vi "Route MT8000A Command.vi"(8 "error in (no error)":errorcluster caption="에러 입력(에러 없음)", 10 "문자열":string, 11 "Instrument Manager 입력":refnum<class "Instrument Manager.lvclass">) -> (0 "error out":errorcluster caption="에러 출력", 3 "Instrument Manager 출력":refnum<class "Instrument Manager.lvclass">)   [LabVIEW 2023, in "Instrument Manager.lvclass"]
uses:
  Instrument Manager.lvclass
  <vilib>/regexp/Match Regular Expression.xnode
  Instrument Manager.lvclass/Instrument Manager.ctl
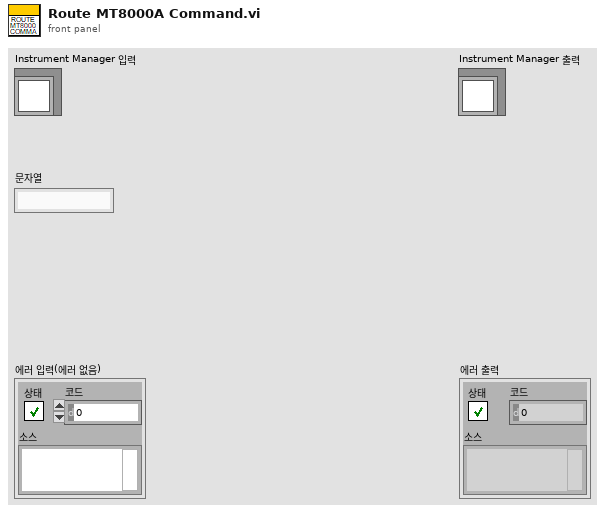
[diagram p1: front panel]
types:
  T1 = typedef "Instrument Manager.lvclass/Connect FSV Params.ctl" = cluster{"type":string, "id":string, "target":string, "command":string, "Params":cluster{"VISA Resource":string}}
  T2 = typedef "NR Call Process Param.ctl" = cluster{"Band":u32, "BandWidth":u32, "Center Channel":u32, "RB Size":i32, "RB Offset":i32, "Modulation":T3, "Max Retry Count":i32, "Wating Time":i32}
  T3 = typedef "ANRITSU Call Box.lvlib/NR Modulation Type.ctl" = enum16{"PI/2 BPSK", "QPSK", "16QAM", "64QAM", "256QAM"}
  T4 = typedef "Instrument Manager.lvclass/Call Process Param.ctl" = cluster{"type":string, "id":string, "target":string, "command":string, "Params":cluster{"Band":u32, "BandWidth":u32, "Center Channel":u32, "RB Size":i32, "RB Offset":i32, "Modulation":string, "Max Retry Count":i32, "Waiting Time":i32}}
  T5 = typedef "NR Call Handover Param.ctl" = cluster{"Band":u32, "BandWidth":u32, "Center Channel":u32, "RB Size":i32, "RB Offset":i32, "Modulation":T3, "Max Retry Count":i32, "Wating Time":i32}
  T6 = typedef "Instrument Manager.lvclass/Call Handover Param.ctl" = cluster{"type":string, "id":string, "target":string, "command":string, "Params":cluster{"Band":u32, "BandWidth":u32, "Center Channel":u32, "RB Size":i32, "RB Offset":i32, "Modulation":string, "Max Retry Count":i32, "Waiting Time":i32}}
  T7 = typedef "NR Handover Param.ctl" = cluster{"Mid Channel":u32, "Band":u32, "BandWidth":u32, "Center Channel":u32, "RB Size":i32, "RB Offset":i32, "Modulation":T3, "Max Retry Count":i32, "Wating Time":i32}
  T8 = typedef "Instrument Manager.lvclass/Handover Param.ctl" = cluster{"type":string, "id":string, "target":string, "command":string, "Params":cluster{"Mid Channel":u32, "Band":u32, "BandWidth":u32, "Center Channel":u32, "RB Size":i32, "RB Offset":i32, "Modulation":string, "Max Retry Count":i32, "Wating Time":i32}}
  T9 = typedef "LTE Call Process Param.ctl" = cluster{"UL Channel":i32, "BandWidth":T10, "RB Offset":i32, "Max Retry Count":i32, "Wating Time":i32}
  T10 = typedef "ANRITSU Call Box.lvlib/LTE Supported BandWidth.ctl" = enum16{"1.4 MHz", "3 MHz", "5 MHz", "10 MHz", "15 MHz", "20 MHz"}
  T11 = typedef "Instrument Manager.lvclass/Call Process Param LTE.ctl" = cluster{"type":string, "id":string, "target":string, "command":string, "Params":cluster{"BandWidth":string, "UL Channel":i32, "RB Offset":i32, "Max Retry Count":i32, "Waiting Time":i32}}
  T12 = typedef "LTE Call Handover Param.ctl" = cluster{"DL Channel":i32, "UL Channel":i32, "BandWidth":T10, "RB Offset":i32, "Max Retry Count":i32, "Wating Time":i32}
  T13 = typedef "Instrument Manager.lvclass/Call Handover Param LTE.ctl" = cluster{"type":string, "id":string, "target":string, "command":string, "Params":cluster{"BandWidth":string, "DL Channel":i32, "UL Channel":i32, "RB Offset":i32, "Max Retry Count":i32, "Waiting Time":i32}}
  T14 = typedef "LTE Handover Param.ctl" = cluster{"Mid Channel":i32, "UL Channel":i32, "BandWidth":T10, "RB Offset":i32, "Max Retry Count":i32, "Wating Time":i32}
  T15 = typedef "Instrument Manager.lvclass/Handover Param LTE.ctl" = cluster{"type":string, "id":string, "target":string, "command":string, "Params":cluster{"BandWidth":string, "Mid Channel":i32, "UL Channel":i32, "RB Offset":i32, "Max Retry Count":i32, "Waiting Time":i32}}
  T16 = typedef "NSA Call Process Param.ctl" = cluster{"Band":u32, "BandWidth":u32, "Center Channel":u32, "RB Size":i32, "RB Offset":i32, "Modulation":T3, "Anchor UL Channel":i32, "Max Retry Count":i32, "Wating Time":i32}
  T17 = typedef "Instrument Manager.lvclass/Call Handover Param NSA.ctl" = cluster{"type":string, "id":string, "target":string, "command":string, "Params":cluster{"Band":u32, "BandWidth":u32, "Center Channel":u32, "RB Size":i32, "RB Offset":i32, "Modulation":string, "Anchor DL Channel":i32, "Max Retry Count":i32, "Waiting Time":i32}}
  T18 = typedef "NSA Call Handover Param.ctl" = cluster{"Band":u32, "BandWidth":u32, "Center Channel":u32, "RB Size":i32, "RB Offset":i32, "Modulation":T3, "Anchor UL Channel":i32, "Max Retry Count":i32, "Wating Time":i32}
  T19 = typedef "Instrument Manager.lvclass/Recall Param.ctl" = cluster{"type":string, "id":string, "target":string, "command":string, "Params":cluster{"Recall Name":string}}
  T20 = typedef "Instrument Manager.lvclass/Default Request.ctl" = cluster{"type":string, "id":string, "target":string, "command":string}
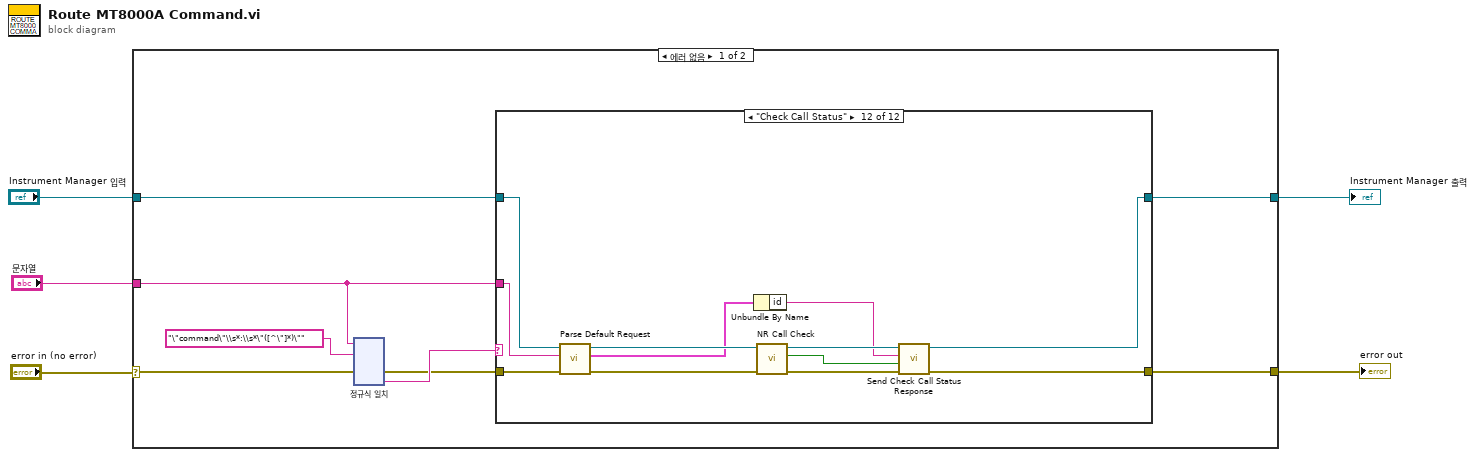
[diagram p0: block diagram]
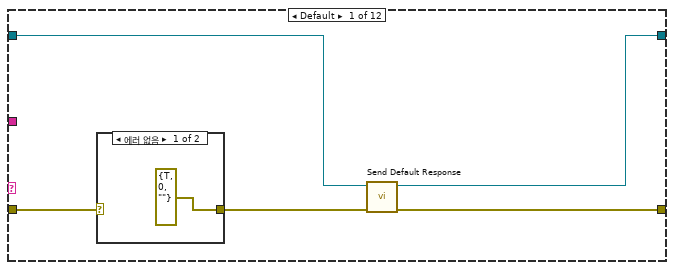
[diagram p2: hidden frame]
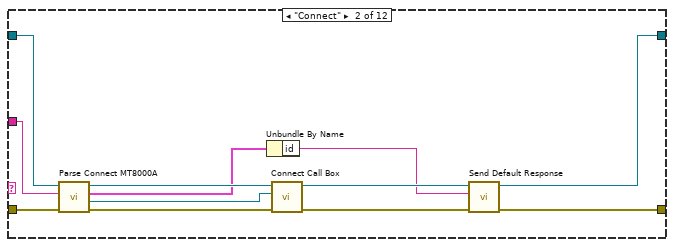
[diagram p4: hidden frame]
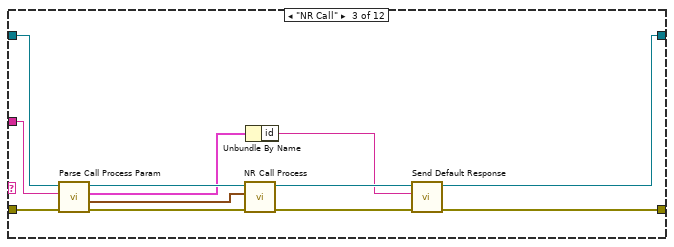
[diagram p5: hidden frame]
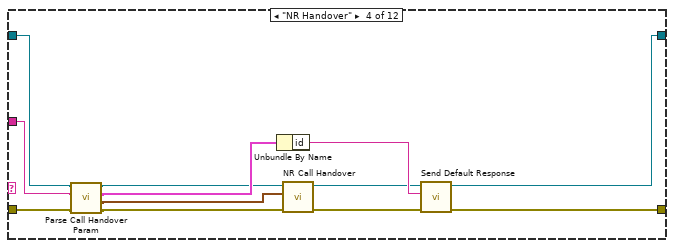
[diagram p6: hidden frame]
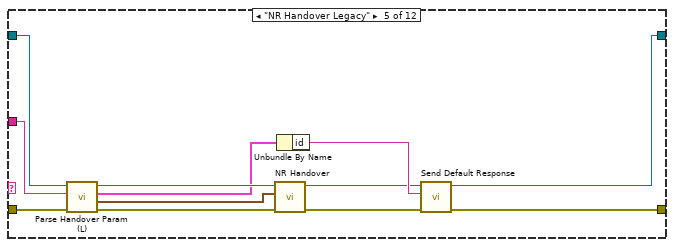
[diagram p7: hidden frame]
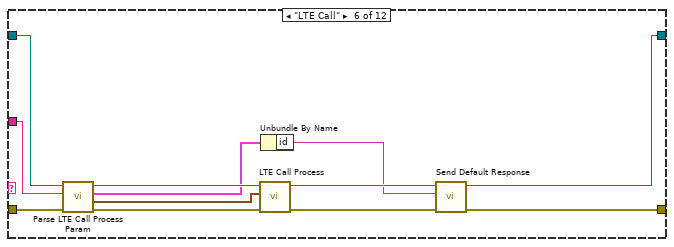
[diagram p8: hidden frame]
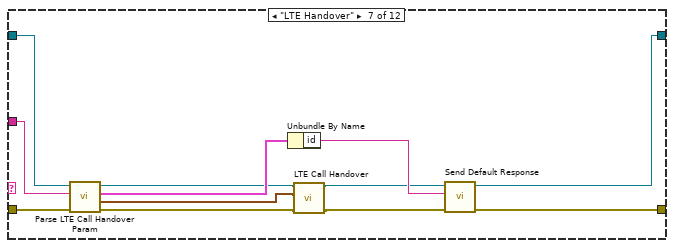
[diagram p9: hidden frame]
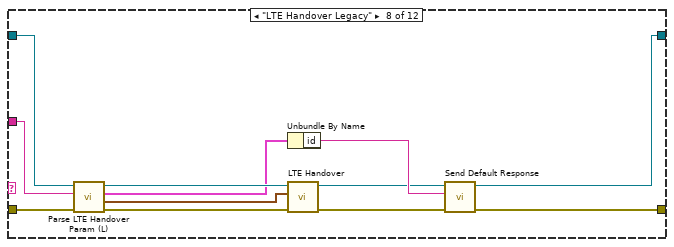
[diagram p10: hidden frame]
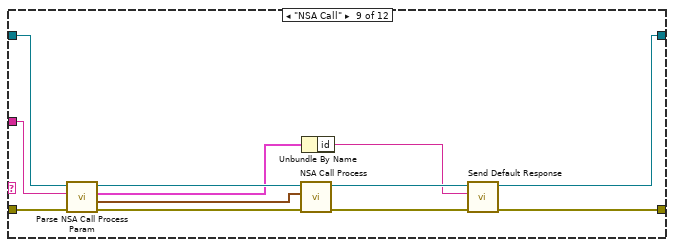
[diagram p11: hidden frame]
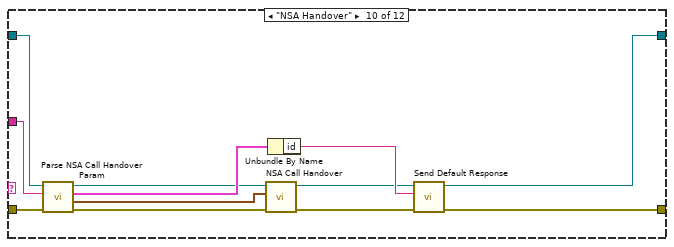
[diagram p12: hidden frame]
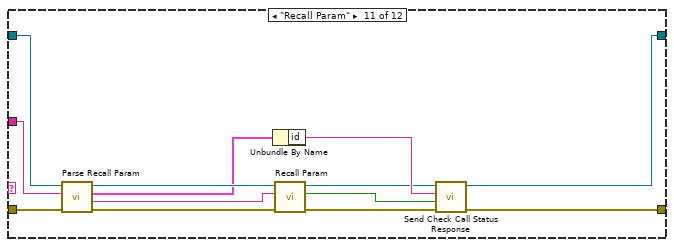
[diagram p13: hidden frame]
diagram:
  n1 = case shown="에러 없음" "error in (no error)" {
    selector: "error in (no error)" -> [w13 w274]
    tunnel: [w7 w274] -> w4
    tunnel: [w6 w273] -> w2
    tunnel: "Instrument Manager 입력" -> [w8 w273]
    tunnel: "문자열" -> [w9 _]
    frame No Error {
      n2 = xnode "정규식 일치"("입력 문자열"=w9, "정규식"="\"command\"\\s*:\\s*\"([^\"]*)\"", "에러 입력"=w13) -> ("에러 출력"=w10:errorcluster, "부분 일치 1"=w11:string)  [unwired: 3 in, 4 out]
      n3 = case shown="\"Check Call Status\"" w11 {
        tunnel: w10 -> [w17 w31 w44 w51 w68 w80 w85 w104 w116 w127 w141 w146]
        tunnel: w9 -> [_ w32 w42 w52 w64 w78 w86 w103 w113 w118 w138 w147]
        tunnel: w8 -> [w15 w30 w43 w53 w63 w79 w87 w102 w114 w119 w139 w148]
        tunnel: [w16 w24 w36 w56 w65 w75 w91 w95 w115 w125 w133 w150] -> w7
        tunnel: [w14 w21 w33 w54 w57 w71 w90 w93 w112 w124 w129 w149] -> w6
        frame Default {
          n4 = case shown="에러 없음" w17 {
            selector: w17 -> [_ w20]
            tunnel: [errorcluster {"status"=TRUE, "code"=0, "source"=""} ("error IO") w20] -> w18
            frame No Error {
            }
            frame Error {
            }
          }
          n5 = call "Send Default Response.vi"("error in (no error)"=w18, "Instrument Manager 입력"=w15) -> ("error out"=w16:errorcluster, "Instrument Manager 출력"=w14:refnum<class "Instrument Manager.lvclass">)  [unwired: 8 in]
        }
        frame "Connect" {
          n6 = call "Parse Connect MT8000A.vi"("error in (no error)"=w31, "JSON string"=w32, "Instrument Manager 입력"=w30) -> ("error out"=w28:errorcluster, "VISA 리소스 이름"=w29:refnum<visa-resource-name>, "Connect FSV Param"=w23:T1, "Instrument Manager 출력"=w27:refnum<class "Instrument Manager.lvclass">)  [unwired: 5 in]
          n7 = Unbundle By Name(w23) -> ("id"=w22:string)
          n8 = call "Connect Call Box.vi"("error in (no error)"=w28, "VISA Address"=w29, "Instrument Manager 입력"=w27) -> ("error out"=w25:errorcluster, "Instrument Manager 출력"=w26:refnum<class "Instrument Manager.lvclass">)  [unwired: 7 in]
          n9 = call "Send Default Response.vi"("error in (no error)"=w25, "id"=w22, "Instrument Manager 입력"=w26) -> ("error out"=w24:errorcluster, "Instrument Manager 출력"=w21:refnum<class "Instrument Manager.lvclass">)  [unwired: 7 in]
        }
        frame "NR Call" {
          n10 = call "Parse Call Process Param.vi"("error in (no error)"=w44, "JSON string"=w42, "Instrument Manager 입력"=w43) -> ("error out"=w40:errorcluster, 1:"NR Call Process Param"=w41:T2, 2:"NR Call Process Param"=w38:T4, "Instrument Manager 출력"=w39:refnum<class "Instrument Manager.lvclass">)  [unwired: 5 in]
          n11 = call "NR Call Process.vi"("error in (no error)"=w40, "NR Call Process Param"=w41, "Instrument Manager 입력"=w39) -> ("error out"=w37:errorcluster, "Instrument Manager 출력"=w35:refnum<class "Instrument Manager.lvclass">)  [unwired: 7 in]
          n12 = Unbundle By Name(w38) -> ("id"=w34:string)
          n13 = call "Send Default Response.vi"("error in (no error)"=w37, "id"=w34, "Instrument Manager 입력"=w35) -> ("error out"=w36:errorcluster, "Instrument Manager 출력"=w33:refnum<class "Instrument Manager.lvclass">)  [unwired: 7 in]
        }
        frame "NR Handover" {
          n14 = call "Parse Call Handover Param.vi"("error in (no error)"=w51, "JSON string"=w52, "Instrument Manager 입력"=w53) -> ("error out"=w45:errorcluster, "NR Call Handover Param"=w46:T5, "Call Handover Param"=w50:T6, "Instrument Manager 출력"=w47:refnum<class "Instrument Manager.lvclass">)  [unwired: 5 in]
          n15 = Unbundle By Name(w50) -> ("id"=w55:string)
          n16 = call "NR Call Handover.vi"("error in (no error)"=w45, "NR Call Handover Param"=w46, "Instrument Manager 입력"=w47) -> ("error out"=w48:errorcluster, "Instrument Manager 출력"=w49:refnum<class "Instrument Manager.lvclass">)  [unwired: 7 in]
          n17 = call "Send Default Response.vi"("error in (no error)"=w48, "id"=w55, "Instrument Manager 입력"=w49) -> ("error out"=w56:errorcluster, "Instrument Manager 출력"=w54:refnum<class "Instrument Manager.lvclass">)  [unwired: 7 in]
        }
        frame "NR Handover Legacy" {
          n18 = call "Parse Handover Param (L).vi"("error in (no error)"=w68, "JSON string"=w64, "Instrument Manager 입력"=w63) -> ("error out"=w67:errorcluster, "NR Call Handover Param"=w61:T7, "Call Handover Param"=w60:T8, "Instrument Manager 출력"=w62:refnum<class "Instrument Manager.lvclass">)  [unwired: 5 in]
          n19 = call "NR Handover.vi"("error in (no error)"=w67, "NR Call Handover Param"=w61, "Instrument Manager 입력"=w62) -> ("error out"=w66:errorcluster, "Instrument Manager 출력"=w58:refnum<class "Instrument Manager.lvclass">)  [unwired: 7 in]
          n20 = Unbundle By Name(w60) -> ("id"=w59:string)
          n21 = call "Send Default Response.vi"("error in (no error)"=w66, "id"=w59, "Instrument Manager 입력"=w58) -> ("error out"=w65:errorcluster, "Instrument Manager 출력"=w57:refnum<class "Instrument Manager.lvclass">)  [unwired: 7 in]
        }
        frame "LTE Call" {
          n22 = call "Parse LTE Call Process Param.vi"("error in (no error)"=w80, "JSON string"=w78, "Instrument Manager 입력"=w79) -> ("error out"=w77:errorcluster, "LTE Call Process Param"=w72:T9, "Call Process Param LTE"=w70:T11, "Instrument Manager 출력"=w74:refnum<class "Instrument Manager.lvclass">)  [unwired: 5 in]
          n23 = call "LTE Call Process.vi"("error in (no error)"=w77, "LTE Call Process Param"=w72, "Instrument Manager 입력"=w74) -> ("error out"=w76:errorcluster, "Instrument Manager 출력"=w73:refnum<class "Instrument Manager.lvclass">)  [unwired: 7 in]
          n24 = Unbundle By Name(w70) -> ("id"=w69:string)
          n25 = call "Send Default Response.vi"("error in (no error)"=w76, "id"=w69, "Instrument Manager 입력"=w73) -> ("error out"=w75:errorcluster, "Instrument Manager 출력"=w71:refnum<class "Instrument Manager.lvclass">)  [unwired: 7 in]
        }
        frame "LTE Handover" {
          n26 = call "Parse LTE Call Handover Param.vi"("error in (no error)"=w85, "JSON string"=w86, "Instrument Manager 입력"=w87) -> ("error out"=w84:errorcluster, "LTE Call Handover Param"=w83:T12, "Call Process Param LTE"=w82:T13, "Instrument Manager 출력"=w81:refnum<class "Instrument Manager.lvclass">)  [unwired: 5 in]
          n27 = Unbundle By Name(w82) -> ("id"=w92:string)
          n28 = call "LTE Call Handover.vi"("error in (no error)"=w84, "LTE Call Handover Param"=w83, "Instrument Manager 입력"=w81) -> ("error out"=w88:errorcluster, "Instrument Manager 출력"=w89:refnum<class "Instrument Manager.lvclass">)  [unwired: 7 in]
          n29 = call "Send Default Response.vi"("error in (no error)"=w88, "id"=w92, "Instrument Manager 입력"=w89) -> ("error out"=w91:errorcluster, "Instrument Manager 출력"=w90:refnum<class "Instrument Manager.lvclass">)  [unwired: 7 in]
        }
        frame "LTE Handover Legacy" {
          n30 = call "Parse LTE Handover Param (L).vi"("error in (no error)"=w104, "JSON string"=w103, "Instrument Manager 입력"=w102) -> ("error out"=w101:errorcluster, "LTE Call Handover Param"=w100:T14, "Call Process Param LTE"=w98:T15, "Instrument Manager 출력"=w99:refnum<class "Instrument Manager.lvclass">)  [unwired: 5 in]
          n31 = Unbundle By Name(w98) -> ("id"=w97:string)
          n32 = call "LTE Handover.vi"("error in (no error)"=w101, "LTE Call Handover Param"=w100, "Instrument Manager 입력"=w99) -> ("error out"=w96:errorcluster, "Instrument Manager 출력"=w94:refnum<class "Instrument Manager.lvclass">)  [unwired: 7 in]
          n33 = call "Send Default Response.vi"("error in (no error)"=w96, "id"=w97, "Instrument Manager 입력"=w94) -> ("error out"=w95:errorcluster, "Instrument Manager 출력"=w93:refnum<class "Instrument Manager.lvclass">)  [unwired: 7 in]
        }
        frame "NSA Call" {
          n34 = call "Parse NSA Call Process Param.vi"("error in (no error)"=w116, "JSON string"=w113, "Instrument Manager 입력"=w114) -> ("error out"=w111:errorcluster, "NSA Call Process Param"=w109:T16, "Call Handover Param LTE"=w106:T17, "Instrument Manager 출력"=w108:refnum<class "Instrument Manager.lvclass">)  [unwired: 5 in]
          n35 = call "NSA Call Process.vi"("error in (no error)"=w111, "NSA Call Process Param"=w109, "Instrument Manager 입력"=w108) -> ("error out"=w110:errorcluster, "Instrument Manager 출력"=w107:refnum<class "Instrument Manager.lvclass">)  [unwired: 7 in]
          n36 = Unbundle By Name(w106) -> ("id"=w105:string)
          n37 = call "Send Default Response.vi"("error in (no error)"=w110, "id"=w105, "Instrument Manager 입력"=w107) -> ("error out"=w115:errorcluster, "Instrument Manager 출력"=w112:refnum<class "Instrument Manager.lvclass">)  [unwired: 7 in]
        }
        frame "NSA Handover" {
          n38 = call "Parse NSA Call Handover Param.vi"("error in (no error)"=w127, "JSON string"=w118, "Instrument Manager 입력"=w119) -> ("error out"=w128:errorcluster, "NSA Call Handover Param"=w121:T18, "Call Handover Param LTE"=w123:T17, "Instrument Manager 출력"=w120:refnum<class "Instrument Manager.lvclass">)  [unwired: 5 in]
          n39 = call "NSA Call Handover.vi"("error in (no error)"=w128, "NSA Call Handover Param"=w121, "Instrument Manager 입력"=w120) -> ("error out"=w126:errorcluster, "Instrument Manager 출력"=w117:refnum<class "Instrument Manager.lvclass">)  [unwired: 7 in]
          n40 = Unbundle By Name(w123) -> ("id"=w122:string)
          n41 = call "Send Default Response.vi"("error in (no error)"=w126, "id"=w122, "Instrument Manager 입력"=w117) -> ("error out"=w125:errorcluster, "Instrument Manager 출력"=w124:refnum<class "Instrument Manager.lvclass">)  [unwired: 7 in]
        }
        frame "Recall Param" {
          n42 = call "Parse Recall Param.vi"("error in (no error)"=w141, "JSON string"=w138, "Instrument Manager 입력"=w139) -> ("error out"=w140:errorcluster, "Recall Name"=w135:string, "Recall Param"=w136:T19, "Instrument Manager 출력"=w137:refnum<class "Instrument Manager.lvclass">)  [unwired: 5 in]
          n43 = Unbundle By Name(w136) -> ("id"=w131:string)
          n44 = call "Recall Param.vi"("error in (no error)"=w140, "Recall Name"=w135, "Instrument Manager 입력"=w137) -> ("error out"=w134:errorcluster, "Connected?"=w132:bool, "Instrument Manager 출력"=w130:refnum<class "Instrument Manager.lvclass">)  [unwired: 6 in]
          n45 = call "Send Check Call Status Response.vi"("error in (no error)"=w134, "connected"=w132, "id"=w131, "Instrument Manager 입력"=w130) -> ("error out"=w133:errorcluster, "Instrument Manager 출력"=w129:refnum<class "Instrument Manager.lvclass">)  [unwired: 6 in]
        }
        frame "Check Call Status" {
          n46 = call "Parse Default Request.vi"("error in (no error)"=w146, "JSON string"=w147, "Instrument Manager 입력"=w148) -> ("error out"=w145:errorcluster, "Default Request"=w143:T20, "Instrument Manager 출력"=w144:refnum<class "Instrument Manager.lvclass">)  [unwired: 6 in]
          n47 = Unbundle By Name(w143) -> ("id"=w142:string)
          n48 = call "NR Call Check.vi"("error in (no error)"=w145, "Instrument Manager 입력"=w144) -> ("error out"=w152:errorcluster, "Connected?"=w153:bool, "Instrument Manager 출력"=w151:refnum<class "Instrument Manager.lvclass">)  [unwired: 7 in]
          n49 = call "Send Check Call Status Response.vi"("error in (no error)"=w152, "connected"=w153, "id"=w142, "Instrument Manager 입력"=w151) -> ("error out"=w150:errorcluster, "Instrument Manager 출력"=w149:refnum<class "Instrument Manager.lvclass">)  [unwired: 6 in]
        }
      }
    }
    frame Error {
    }
  }
  "error out" <- w4
  "Instrument Manager 출력" <- w2
